vi "VIH Project Tree - Relink Item Rule to New Path (w descendants).vi"(8 "error in":errorcluster, 9 "Old Item Path":path, 10 "New Item Path":path, 11 "Project Tree":T1) -> (0 "error out":errorcluster, 1 "dup Old Item Path":path, 2 "dup New Item Path":path, 3 "dup Project Tree":T1)   [LabVIEW 2014]
doc: "::: VI Helpeks :::\nCopyright (c) 2000-2026 Konstantin Shifershteyn. All rights reserved."
uses:
  VIH Project Tree Typedef - Tree Refnum.ctl
panel:
  # "VI Helpeks\nCopyright (c) 2012-2026 Konstantin Shifershteyn"
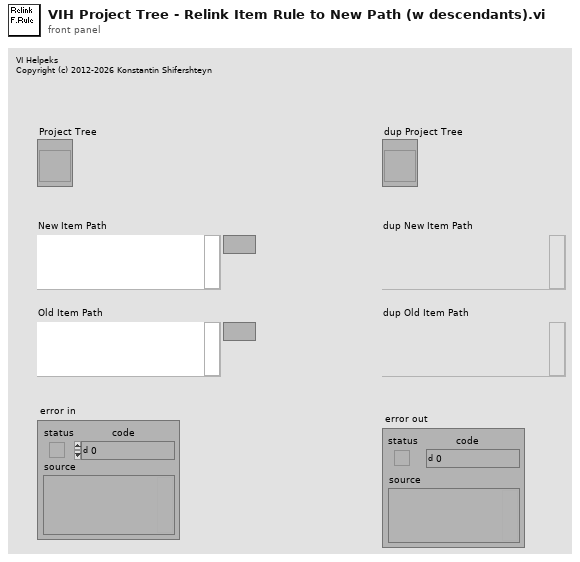
[diagram p1: front panel]
types:
  T1 = typedef "VIH Project Tree Typedef - Tree Refnum.ctl" = refnum<vi>
  T2 = enum16{"get", "get all", "set", "Init", "delete", "rename"}
  T3 = typedef "VIH HelpGen Typedef - Palette - Item Type Enum.ctl" = enum32{"<Invalid>", "<unknown>", "VI", "Menu", "LV Func", "Express VI", "Poly VI", "CTL", "HTML"}
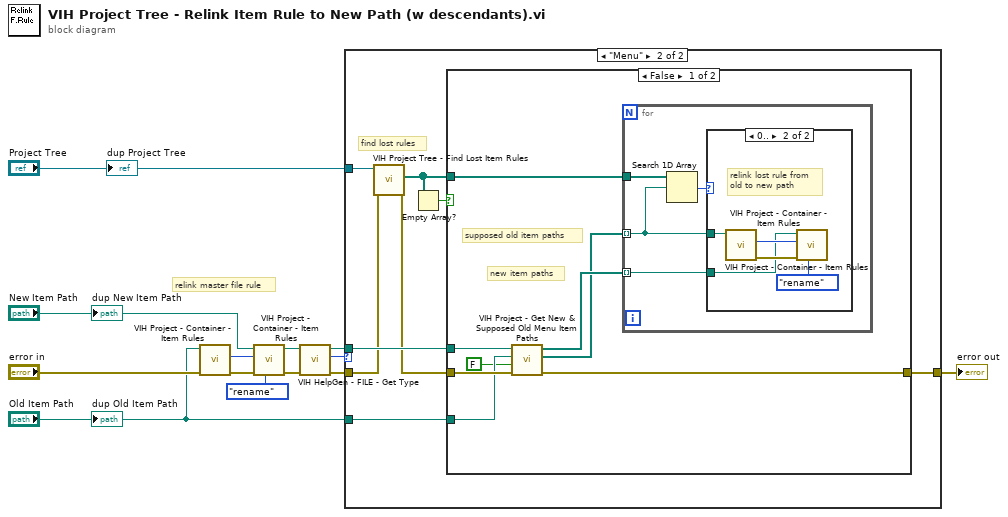
[diagram p0: block diagram]
diagram:
  # "relink master file rule"
  n1 = call "VIH Project - Container - Item Rules.vi"("error in"="error in", "Item Path"="Old Item Path") -> ("error out"=w8:errorcluster, "Item Idx out"=w11:i32)  [unwired: 5 in, 3 out]
  n2 = call "VIH Project - Container - Item Rules.vi"("cmd (get)"=T2."rename", "error in"=w8, "Item Idx (-1)"=w11, "Item Path"="New Item Path") -> ("error out"=w7:errorcluster, "Item Path out"=w9:path)  [unwired: 3 in, 3 out]
  n3 = call "VIH HelpGen - FILE - Get Type.vi"("error in"=w7, "File Path"=w9) -> ("error out"=w6:errorcluster, "File Type"=w13:T3, "dup File Path"=w12:path)  [unwired: 7 in]
  n4 = case shown="\"Menu\"" w13 {
    tunnel: w12 -> [_ w22]
    tunnel: w6 -> [w14 w21]
    tunnel: "Project Tree" -> [_ w19]
    tunnel: [w14 w18] -> w4
    tunnel: "Old Item Path" -> [_ w15]
    frame Default {
    }
    frame "Menu" {
      # "find lost rules"
      n5 = call "VIH Project Tree - Find Lost Item Rules.vi"("error in"=w21, "Project Tree"=w19) -> ("error out"=w20:errorcluster, "Lost Rules (Owner Paths)"=w16:path[])  [unwired: 7 in, 1 out]
      n6 = Empty Array?(array=w16) -> (empty?=w17:bool)
      n7 = case shown="False" w17 {
        tunnel: w22 -> [w29 _]
        tunnel: w20 -> [w28 w40]
        tunnel: [w27 w40] -> w18
        tunnel: w16 -> [w30 _]
        tunnel: w15 -> [w26 _]
        frame False {
          # "new item paths"
          # "supposed old item paths"
          n8 = call "VIH Project - Get New & Supposed Old Menu Item Paths.vi"("error in"=w28, "Test File Type (T)"=FALSE, "old Menu Path"=w26, "new Menu Path"=w29) -> ("error out"=w27:errorcluster, "Supposed Old Item Paths"=w23:path[], "New Item Paths"=w24:path[])  [unwired: 5 in]
          n9 = for {
            tunnel: w24 -> [w32] mode=indexing
            tunnel: w30 -> [w34]
            tunnel: w23 -> [w31] mode=indexing
            n10 = Search 1D Array(1D array=w34, element=w31) -> (index of element=w33:i32)  [unwired: 1 in]
            n11 = case shown="0.." w33 {
              tunnel: w31 -> [_ w36]
              tunnel: w32 -> [_ w35]
              frame ..-1 {
              }
              frame 0.. {
                # "relink lost rule from\nold to new path"
                n12 = call "VIH Project - Container - Item Rules.vi"("Item Path"=w36) -> ("error out"=w37:errorcluster, "Item Idx out"=w39:i32)  [unwired: 6 in, 3 out]
                n13 = call "VIH Project - Container - Item Rules.vi"("cmd (get)"=T2."rename", "error in"=w37, "Item Idx (-1)"=w39, "Item Path"=w35) -> ()  [unwired: 3 in, 5 out]
              }
            }
          }
        }
        frame True {
        }
      }
    }
  }
  "error out" <- w4
  "dup Project Tree" <- "Project Tree"
  "dup New Item Path" <- "New Item Path"
  "dup Old Item Path" <- "Old Item Path"
